vi "lvmcp_libadd.vi"(7 "Type":string, 9 "Name":string, 10 "item":path, 11 "library":path) -> (0 "error out":errorcluster)   [LabVIEW 2015]
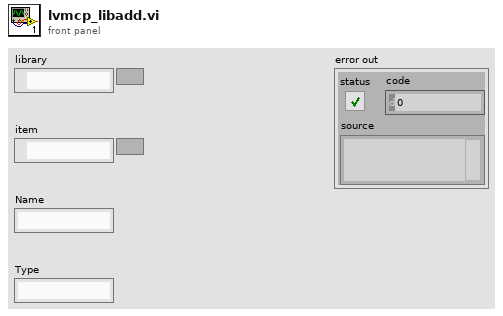
[diagram p1: front panel]
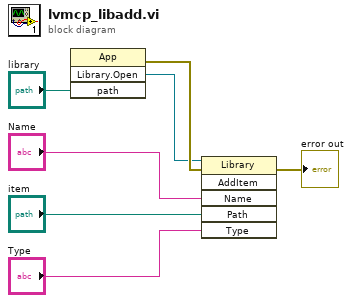
[diagram p0: block diagram]
diagram:
  n1 = invoke class="App" method="Library.Open"("path"="library") -> (error out=w6:errorcluster, "Open Library"=w1:refnum<vi>)  [unwired: 3 in, 2 out]
  n2 = invoke class="Library" method="AddItem"(reference=w1, error in=w6, "Name"="Name", "Path"="item", "Type"="Type") -> (error out=→"error out":errorcluster)  [unwired: 1 in, 5 out]
